vi "Resource URI.vi"(10 "derived uri":string, 11 "uri":string) -> (3 "uri out":string)   [LabVIEW 2020, in "MCP Server.lvlib"]
doc: "Chooses the uri under which Add Resource (File).vi lists a resource and resources/read finds it: uri when it is not empty, otherwise the uri derived from the file name (labview://<MCP name>). The uri is used exactly as given; nothing is checked or encoded."
uses:
  MCP Server.lvlib
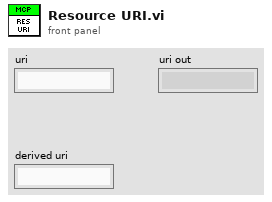
[diagram p1: front panel]
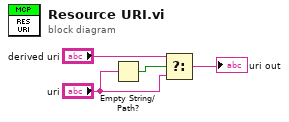
[diagram p0: block diagram]
diagram:
  n1 = Empty String/Path?(string/path="uri") -> (empty?=w4:bool)
  n2 = Select(t="derived uri", s=w4, f="uri") -> (s? t:f=→"uri out":string)
